vi "measure BT Frequency Separation Step3.vi"(8 "error in (no error)":errorcluster, 10 "Packet BW":dbl, 11 "SA Measurement in":refnum<class "SA Measurement.lvclass">) -> (0 "error out":errorcluster, 3 "SA Measurement out":refnum<class "SA Measurement.lvclass">)   [LabVIEW 2023, in "Spectrum Analyzer.lvlib" / "SA Measurement.lvclass"]
uses:
  SA Measurement.lvclass
  SA Measurement.lvclass/SA Measurement.ctl
  Interface_Spectrum/Interface_Spectrum.lvclass
  TYPE DEFINITION/TYPE Marker Control Mode.ctl
  Spectrum Analyzer.lvlib
  TYPE DEFINITION/TYPE Marker Peak Search Type.ctl
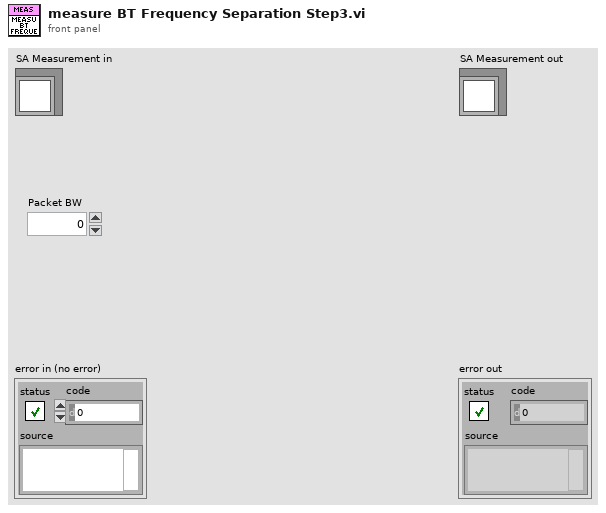
[diagram p1: front panel]
types:
  T1 = typedef "Spectrum Analyzer.lvlib/TYPE Marker Control Mode.ctl" = enum16{"Normal", "Delta", "Off"}
  T2 = typedef "Spectrum Analyzer.lvlib/TYPE Marker Peak Search Type.ctl" = enum16{"Max", "Next Peak"}
  T3 = typedef "Spectrum Analyzer.lvlib/TYPE Marker Value.ctl" = cluster{"X-axis":dbl, "Y-axis":dbl}
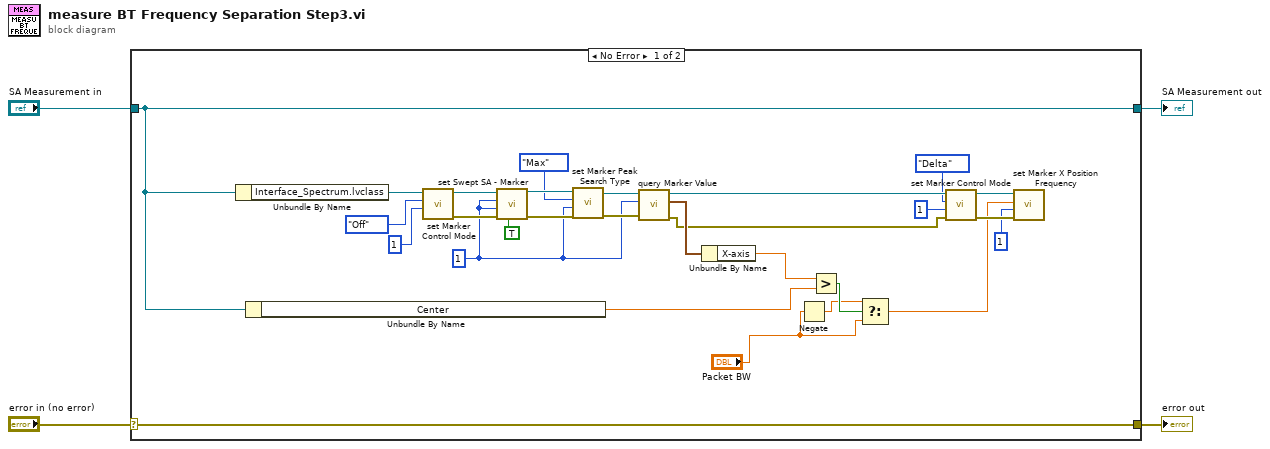
[diagram p0: block diagram]
diagram:
  n1 = case shown="No Error" "error in (no error)" {
    selector: "error in (no error)" -> [w32 w34]
    tunnel: [w32 w34] -> w3
    tunnel: [w8 w33] -> w1
    tunnel: "SA Measurement in" -> [w8 w33]
    frame No Error {
      w20 = 1 ("Index")
      n2 = Unbundle By Name(w8) -> ("Interface_Spectrum.lvclass"=w31:refnum<class "Interface_Spectrum.lvclass">)
      n3 = Unbundle By Name(w8) -> ("Center"=w7:dbl)
      n4 = call-dynamic "set Marker Control Mode.vi"("Marker Index"=1, "Marker Mode"=TYPE_Marker_Control_Mode."Off", "Interface_Spectrum in"=w31) -> ("error out"=w23:errorcluster, "Interface_Spectrum out"=w24:refnum<class "Interface_Spectrum.lvclass">)  [unwired: 7 in]
      n5 = call-dynamic "set Swept SA - Marker.vi"("On?"=TRUE, "error in (no error)"=w23, "trace"=w20, "Index"=w20, "Interface_Spectrum in"=w24) -> ("error out"=w26:errorcluster, "Interface_Spectrum out"=w27:refnum<class "Interface_Spectrum.lvclass">)  [unwired: 5 in]
      n6 = call-dynamic "set Marker Peak Search Type.vi"("error in (no error)"=w26, "Marker Index"=w20, "Peak Search Type"=TYPE_Marker_Peak_Search_Type."Max", "Interface_Spectrum in"=w27) -> ("error out"=w21:errorcluster, "Interface_Spectrum out"=w22:refnum<class "Interface_Spectrum.lvclass">)  [unwired: 6 in]
      n7 = call-dynamic "query Marker Value.vi"("error in (no error)"=w21, "Marker Index"=w20, "Interface_Spectrum in"=w22) -> ("error out"=w13:errorcluster, "Marker Value"=w19:T3, "Interface_Spectrum out"=w16:refnum<class "Interface_Spectrum.lvclass">)  [unwired: 6 in]
      n8 = Unbundle By Name(w19) -> ("X-axis"=w18:dbl)
      n9 = Negate(x="Packet BW") -> (-x=w5:dbl)
      n10 = Greater?(x=w18, y=w7) -> (0:w17:bool)
      n11 = Select(t=w5, s=w17, f="Packet BW") -> (s? t:f=w9:dbl)
      n12 = call-dynamic "set Marker Control Mode.vi"("error in (no error)"=w13, "Marker Index"=1, "Marker Mode"=TYPE_Marker_Control_Mode."Delta", "Interface_Spectrum in"=w16) -> ("error out"=w11:errorcluster, "Interface_Spectrum out"=w12:refnum<class "Interface_Spectrum.lvclass">)  [unwired: 6 in]
      n13 = call-dynamic "set Marker X Position Frequency.vi"("error in (no error)"=w11, "Index"=1, "X Position Frequency (Hz)"=w9, "Interface_Spectrum in"=w12) -> ()  [unwired: 6 in, 2 out]
    }
    frame Error {
    }
  }
  "error out" <- w3
  "SA Measurement out" <- w1
